vi "Measurement Logic.vi"() -> ()   [LabVIEW 2021, in "NIScopeAcquireWaveform.lvlib"]
uses:
  NIScopeAcquireWaveform.lvlib
  Measurement Results.ctl
  <vilib>/Plug-In SDKs/Measurements/Measure Call Context/Measure Call Context.lvclass
  Measurement Configuration.ctl
  <instrlib>/niScope/Controls/niScope vertical coupling.ctl
  <instrlib>/niScope/Controls/niScope trigger slope.ctl
  <vilib>/Plug-In SDKs/Sessions/niScope/Initialize Sessions - 1Sess.vi
  <instrlib>/niScope/Configure/Trigger/niScope Configure Trigger Edge.vi
  <instrlib>/niScope/Acquire/Fetch/niScope Fetch.vi
  <extravilib>/ChannelInstances/One Element Stream-bool/Instantiate.vi
  <vilib>/Plug-In SDKs/Clients/Session Management V1/Session Reservation/Session Reservation.lvclass
  <vilib>/Plug-In SDKs/Sessions/niScope/NI Session Management niScope.lvlib
panel:
  in  "measurement configuration":T1={"Measurement Pins"=["PinGroup1"], "Vertical Range"=5.0, "Vertical Coupling"=1, "Input Impedance"=0, "Minimum Sample Rate"=10000000.0, "Minimum Record Length"=40000, "Trigger Pin"="Pin1", "Trigger Level"=0.5, "Trigger Slope"=0, "Timeout"=5.0, "Trigger Coupling"=1} {"Input Impedance" items=["1 mega ohm"=0, "50 ohms"=2]; "Trigger Coupling" items=["AC"=0, "DC"=1, "HF Reject"=3, "LF Reject"=4, "AC Plus HF Reject"=1001]; "Trigger Slope" items=["Positive", "Negative"]; "Vertical Coupling" items=["AC", "DC", "Ground"]}
  out "measure call context out":refnum<class "Measure Call Context.lvclass">
  in  "measure call context in":refnum<class "Measure Call Context.lvclass">
  out "measurement results":T4
  out "error out":errorcluster
  in  "error in":errorcluster
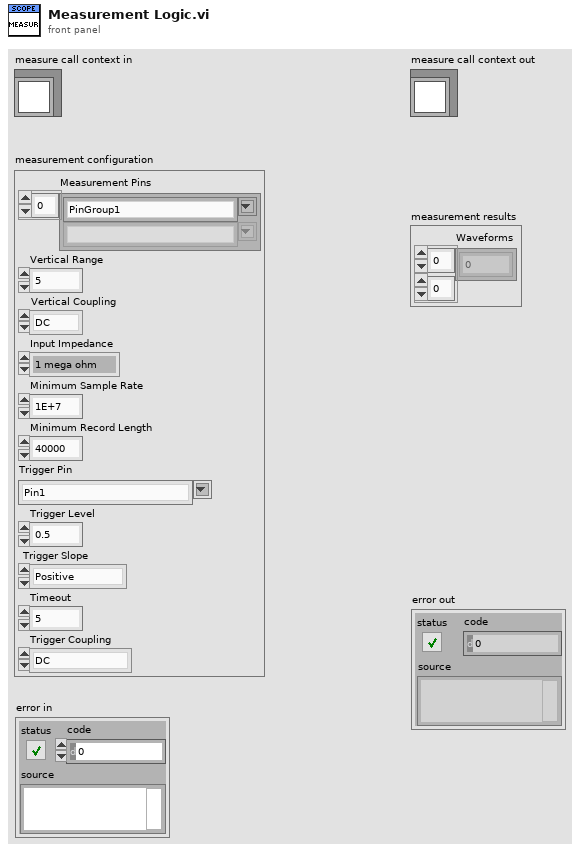
[diagram p1: front panel]
types:
  T1 = typedef "NIScopeAcquireWaveform.lvlib/Measurement Configuration.ctl" = cluster{"Measurement Pins":string[], "Vertical Range":dbl, "Vertical Coupling":T2, "Input Impedance":u32, "Minimum Sample Rate":dbl, "Minimum Record Length":i32, "Trigger Pin":string, "Trigger Level":dbl, "Trigger Slope":T3, "Timeout":dbl, "Trigger Coupling":u32}
  T2 = typedef "niScope vertical coupling.ctl" = i32
  T3 = typedef "niScope trigger slope.ctl" = i32
  T4 = typedef "NIScopeAcquireWaveform.lvlib/Measurement Results.ctl" = cluster{"Waveforms":dbl[][]}
  T5 = typedef "NI Session Management niScope.lvlib/Connection with Session.ctl" = cluster{"connection":T6, "session":refnum<k15>}
  T6 = typedef "NI Session Management V1 Client.lvlib/Session Reservation.lvclass/Connection.ctl" = cluster{"pin or relay name":string, "site":i32, "instrument type id":string, "channel":string}
  T7 = typedef "One Element Stream-bool.lvlib/)Channel.ctl" = refnum<queue>
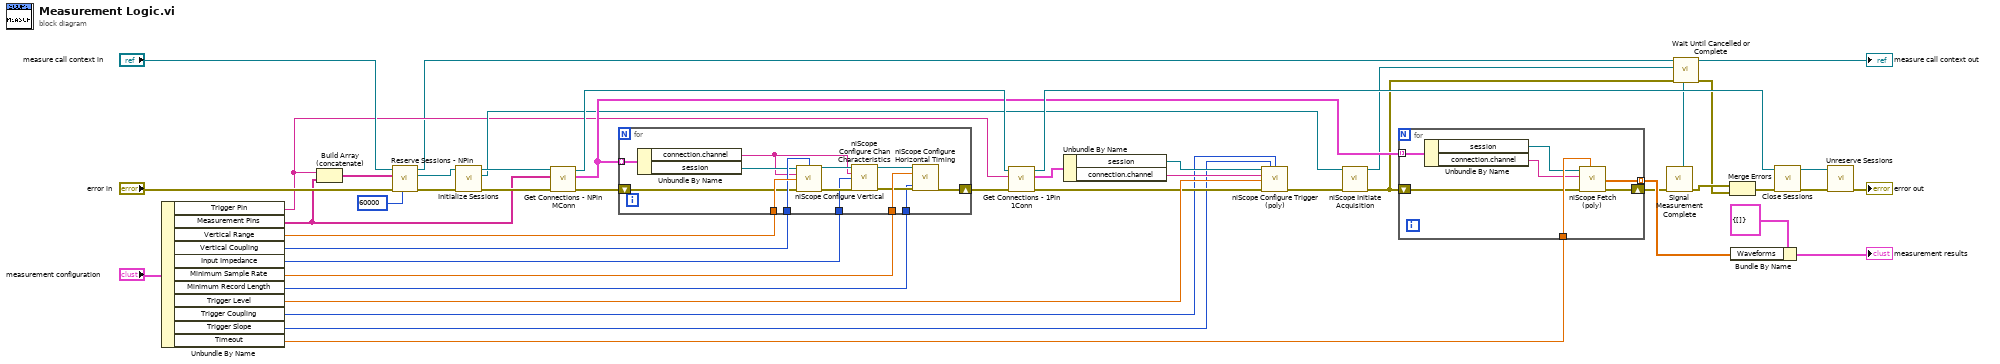
[diagram p0: block diagram]
diagram:
  n1 = Unbundle By Name("measurement configuration") -> ("Trigger Pin"=w15:string, "Measurement Pins"=w16:string[], "Vertical Range"=w40:dbl, "Vertical Coupling"=w38:T2, "Input Impedance"=w34:u32, "Minimum Sample Rate"=w30:dbl, "Minimum Record Length"=w29:i32, "Trigger Level"=w39:dbl, "Trigger Coupling"=w12:u32, "Trigger Slope"=w11:T3, "Timeout"=w37:dbl)
  n2 = Build Array (concatenate)(w15, w16) -> (w14:string[])
  n3 = call <vilib>:"Reserve Sessions - NPin.vi"("timeout (ms)"=60000, "error in"="error in", "pin or relay names"=w14, "measurement context in"="measure call context in") -> ("error out"=w41:errorcluster, "session reservation out"=w42:refnum<class "Session Reservation.lvclass">, "measurement context out"=w8:refnum<class "Measure Call Context.lvclass">)  [unwired: 5 in]
  n4 = call-poly <vilib>:"Initialize Sessions.vi"("error in"=w41, "session reservation in"=w42) -> ("error out"=w33:errorcluster, "session"=w19:refnum<k15>, "session reservation out"=w32:refnum<class "Session Reservation.lvclass">)  [unwired: 6 in, 1 out]
  n5 = call <vilib>:"Get Connections - NPin MConn.vi"("error in"=w33, "pin or relay names"=w16, "session reservation in"=w32) -> ("error out"=w31:errorcluster, "connections"=w21:T5[], "session reservation out"=w26:refnum<class "Session Reservation.lvclass">)  [unwired: 6 in]
  n6 = for {
    tunnel: w40 -> [w59]
    tunnel: w38 -> [w57]
    tunnel: w34 -> [w56]
    shift-right: [w48] -> w28
    shift-left: w31 -> [w55]
    tunnel: w21 -> [w54] mode=indexing
    tunnel: w30 -> [w52]
    tunnel: w29 -> [w50]
    n7 = Unbundle By Name(w54) -> ("connection.channel"=w47:string, "session"=w53:refnum<k15>)
    n8 = call <instrlib>:"niScope Configure Vertical.vi"("instrument handle"=w53, "vertical coupling"=w57, "channels"=w47, "vertical range"=w59, "error in"=w55) -> ("instrument handle out"=w60:refnum<k15>, "error out"=w58:errorcluster)  [unwired: 9 in]
    n9 = call <instrlib>:"niScope Configure Chan Characteristics.vi"("instrument handle"=w60, "channels"=w47, "input impedance"=w56, "error in"=w58) -> ("instrument handle out"=w49:refnum<k15>, "error out"=w51:errorcluster)  [unwired: 10 in]
    n10 = call <instrlib>:"niScope Configure Horizontal Timing.vi"("instrument handle"=w49, "min sample rate"=w52, "error in"=w51, "min record length"=w50) -> ("error out"=w48:errorcluster)  [unwired: 10 in, 1 out]
  }
  n11 = call <vilib>:"Get Connections - 1Pin 1Conn.vi"("error in"=w28, "pin or relay name"=w15, "session reservation in"=w26) -> ("error out"=w27:errorcluster, "connection"=w25:T5, "session reservation out"=w22:refnum<class "Session Reservation.lvclass">)  [unwired: 6 in]
  n12 = Unbundle By Name(w25) -> ("session"=w24:refnum<k15>, "connection.channel"=w23:string)
  n13 = call-poly <instrlib>:"niScope Configure Trigger (poly).vi"("instrument handle"=w24, "trigger slope"=w11, "trigger coupling"=w12, "trigger source"=w23, "trigger level"=w39, "error in"=w27) -> ("error out"=w20:errorcluster)  [unwired: 8 in, 1 out]
  n14 = call <instrlib>:"niScope Initiate Acquisition.vi"("instrument handle"=w19, "error in"=w20) -> ("instrument handle out"=w6:refnum<k15>, "error out"=w3:errorcluster)  [unwired: 12 in]
  n15 = for {
    tunnel: [w67] -> w13 mode=indexing
    tunnel: w37 -> [w66]
    shift-right: [w65] -> w5
    shift-left: w3 -> [w61]
    tunnel: w21 -> [w64] mode=indexing
    n16 = Unbundle By Name(w64) -> ("session"=w63:refnum<k15>, "connection.channel"=w62:string)
    n17 = call-poly <instrlib>:"niScope Fetch (poly).vi"("timeout"=w66, "error in"=w61, "channels"=w62, "instrument handle"=w63) -> ("error out"=w65:errorcluster, "wfm"=w67:dbl[])  [unwired: 4 in, 2 out]
  }
  n18 = call "Signal Measurement Complete.vi"("error in (no error)"=w5) -> ("error out"=w4:errorcluster, "done channel"=w1:T7)  [unwired: 9 in]
  n19 = call "Wait Until Cancelled or Complete.vi"("done channel"=w1, "error in (no error)"=w3, "scope session"=w6, "measure call context in"=w8) -> ("error out"=w2:errorcluster, "neasure call context out"=→"measure call context out":refnum<class "Measure Call Context.lvclass">)  [unwired: 6 in]
  n20 = Merge Errors(w4, w2) -> (w10:errorcluster)
  n21 = Bundle By Name(cluster=T4 {"Waveforms"=[]} ("Measurement Results"), "Waveforms"=w13) -> (→"measurement results":T4)
  n22 = call <vilib>:"Close Sessions.vi"("error in"=w10, "session reservation in"=w22) -> ("error out"=w36:errorcluster, "session reservation out"=w35:refnum<class "Session Reservation.lvclass">)  [unwired: 8 in]
  n23 = call <vilib>:"Unreserve Sessions.vi"("error in"=w36, "session reservation in"=w35) -> ("error out"=→"error out":errorcluster)  [unwired: 9 in]
